vi "ZM-ROOT-helperPanel.vi"(8 "error in":errorcluster, 10 "Event Registration Refnum":refnum<event-registration>, 11 "ZM-ROOT-root in":refnum<class "ZM-ROOT-root.lvclass">) -> (0 "error out":errorcluster)   [LabVIEW 2020, in "ZM-ROOT-root.lvlib" / "ZM-ROOT-root.lvclass"]
doc: "Panel loop of the root, started by Actor Core beside Call Parent; its panel shows the Stop button and the errors list. Stop sends Normal Stop to the root, an error event appends its text to errors, and the stop event ends the loop. Error-handling plan: none yet; on an error the loop ends and sends Normal Stop to its own actor."
uses:
  ZM-ROOT-root.lvclass
  <vilib>/ActorFramework/Stop Msg/Stop Msg.lvclass
  <vilib>/ActorFramework/Message Enqueuer/Message Enqueuer.lvclass
  <vilib>/ActorFramework/Actor/Actor.lvclass
panel:
  in  "Stop":bool
  out "errors":string
  # "To watch the data being sent: in the project, open the virtual folder \"receiver\" and run ZM-receiver.vi (UDP 127.0.0.1:61557)."
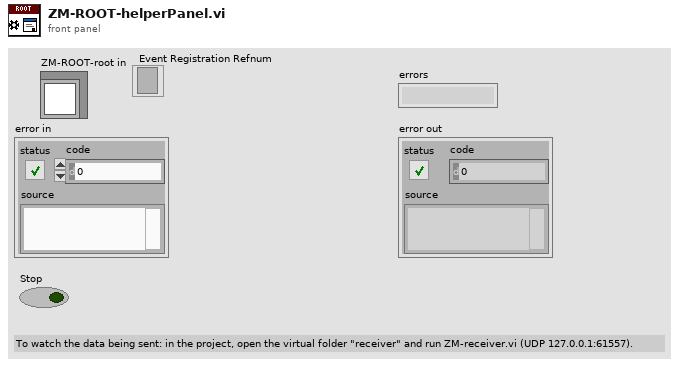
[diagram p1: front panel]
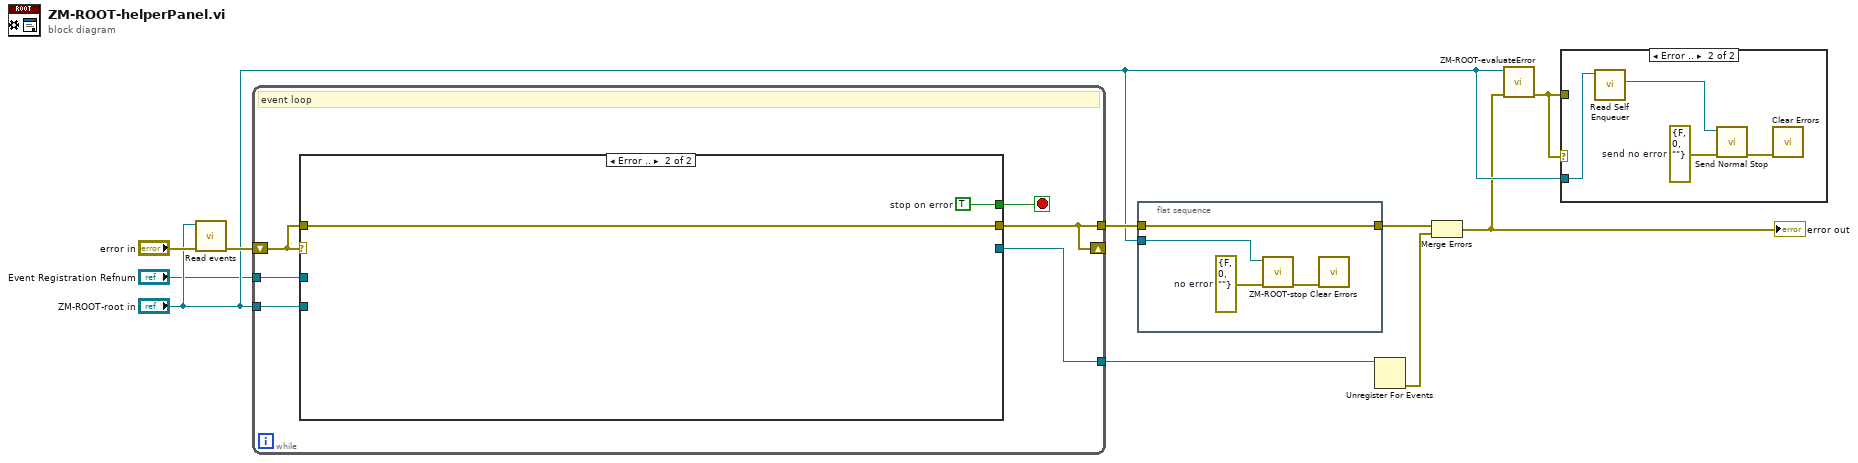
[diagram p0: block diagram]
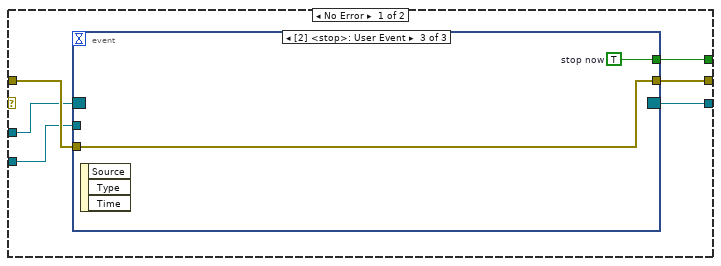
[diagram p3: hidden frame]
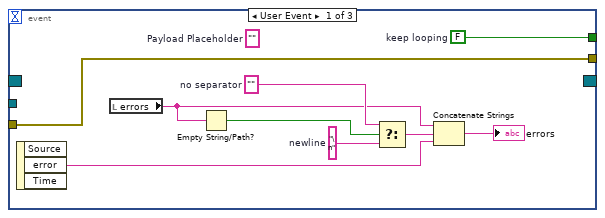
[diagram p4: hidden frame]
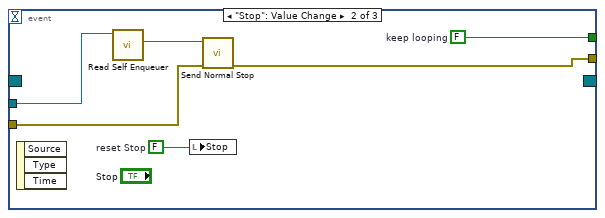
[diagram p5: hidden frame]
diagram:
  n1 = call "Read events.vi"("error in (no error)"="error in", "ZM-ROOT-root in"="ZM-ROOT-root in") -> ("error out"=w9:errorcluster)  [unwired: 7 in, 2 out]
  n2 = while {
    tunnel: "ZM-ROOT-root in" -> [w16]
    shift-right: [w13] -> _
    shift-left: w9 -> [w15]
    tunnel: [w13] -> w8
    tunnel: "Event Registration Refnum" -> [w12]
    tunnel: [w11] -> w2
    stop <- w14 stop-if-true
    # "event loop"
    n3 = case shown="Error .." w15 {
      tunnel: w15 -> [w22 w41]
      tunnel: w16 -> [w21 _]
      tunnel: [w20 w41] -> w13
      tunnel: [w19 w40] -> w14
      tunnel: w12 -> [w18 _]
      tunnel: [w17 _] -> w11
      frame No Error {
        n4 = event shown="[2] <stop>: User Event" {
          selector: w18 -> [_ _ _]
          dyn-events: [_ _ _] -> w17
          timeout: _ -> [_ _ _]
          tunnel: w22 -> [w23 w35 w38]
          tunnel: w21 -> [_ w36 _]
          tunnel: [w24 w33 w39] -> w19
          tunnel: [w23 w32 w38] -> w20
          event User Event {
            w24 = FALSE  # keep looping
            w29 = "\n"  # newline
            w31 = ""  # no separator
            (unwired) ""  # Payload Placeholder
            n5 = event-data() -> ("error"=w26:string)  [unwired: 1 in, 2 out]
            n6 = local read "errors"() -> (w28:string)
            n7 = Empty String/Path?(string/path=w28) -> (empty?=w30:bool)
            n8 = Select(t=w31, s=w30, f=w29) -> (s? t:f=w27:string)
            n9 = Concatenate Strings(w28, w27, w26) -> (→"errors":string)
          }
          event "Stop": Value Change {
            w33 = FALSE  # keep looping
            w37 = FALSE  # reset Stop
            n10 = event-data() -> ()  [unwired: 1 in, 3 out]
            n11 = call <vilib>:"Read Self Enqueuer.vi"("Actor"=w36) -> ("Self Enqueuer"=w34:refnum<class "Message Enqueuer.lvclass">)  [unwired: 10 in]
            n12 = local write "Stop"(w37) -> ()
            n13 = call <vilib>:"Send Normal Stop.vi"("error in (no error)"=w35, "Message Enqueuer"=w34) -> ("error out"=w32:errorcluster)  [unwired: 9 in]
          }
          event User Event {
            w39 = TRUE  # stop now
            n14 = event-data() -> ()  [unwired: 1 in, 3 out]
          }
        }
      }
      frame Error {
        w40 = TRUE  # stop on error
      }
    }
  }
  n15 = flat-sequence {
    tunnel: w8 -> [w42]
    tunnel: "ZM-ROOT-root in" -> [w45]
    tunnel: [w42] -> w7
    frame #0 {
      w44 = errorcluster {"status"=FALSE, "code"=0, "source"=""}  # no error
      n16 = call "ZM-ROOT-stop.vi"("error in (no error)"=w44, "ZM-ROOT-root in"=w45) -> ("error out"=w43:errorcluster)  [unwired: 8 in, 1 out]
      n17 = call <vilib>:"Clear Errors.vi"("error in (no error)"=w43) -> ()  [unwired: 5 in, 2 out]
    }
  }
  n18 = Unregister For Events(event registration refnum=w2) -> (error out=w6:errorcluster)  [unwired: 1 in]
  n19 = Merge Errors(w7, w6) -> (w3:errorcluster)
  "error out" <- w3
  n20 = call "ZM-ROOT-evaluateError.vi"("error in (no error)"=w3, "ZM-ROOT-root in"="ZM-ROOT-root in") -> ("error out"=w4:errorcluster)  [unwired: 7 in, 2 out]
  n21 = case shown="Error .." w4 {
    tunnel: w4 -> [_ _]
    tunnel: "ZM-ROOT-root in" -> [_ w49]
    frame No Error {
    }
    frame Error {
      w48 = errorcluster {"status"=FALSE, "code"=0, "source"=""}  # send no error
      n22 = call <vilib>:"Read Self Enqueuer.vi"("Actor"=w49) -> ("Self Enqueuer"=w47:refnum<class "Message Enqueuer.lvclass">)  [unwired: 10 in]
      n23 = call <vilib>:"Send Normal Stop.vi"("error in (no error)"=w48, "Message Enqueuer"=w47) -> ("error out"=w46:errorcluster)  [unwired: 9 in]
      n24 = call <vilib>:"Clear Errors.vi"("error in (no error)"=w46) -> ()  [unwired: 5 in, 2 out]
    }
  }
